vi "DCIMG to HDF5.vi"(4 "Time points":cluster{"Time Offset":i32, "Max length ":i32}={"Time Offset"=0, "Max length "=2147483647}, 5 "Chunk size":i32[](array[numeric])=[60, 256, 512], 6 "Frames per volume":i32=61, 7 "Channels":T1(array[cluster])=[{"X Offset"=0, "X Length"=512, "Y Offset"=0, "Y Length"=256, "Z Start"=0, "Z End"=60, "Z Stride"=1, "Name"="Far Red"}, {"X Offset"=512, "X Length"=512, "Y Offset"=0, "Y Length"=256, "Z Start"=0, "Z End"=60, "Z Stride"=1, "Name"="Red"}, {"X Offset"=1024, "X Length"=512, "Y Offset"=0, "Y Length"=256, "Z Start"=0, "Z End"=60, "Z Stride"=1, "Name"="Green"}], 8 "error in (no error)":errorcluster, 10 "Output path (*.h5)":path, 11 "Input path (*.dcimg)":path) -> (0 "error out":errorcluster)   [LabVIEW 2020]
uses:
  <vilib>/UPVI/lvhdf5/dataset.llb/LVH5D Operation.ctl
  <vilib>/Utility/miscctls.llb/LVRectTypeDef.ctl
  <vilib>/UPVI/lvhdf5/group.llb/H5G_obj_t.ctl
  <vilib>/Analysis/1siggen.llb/Ramp Pattern by Delta.vi
  <vilib>/UPVI/lvhdf5/utility.llb/Select HDF5 Dialog.vi
  <vilib>/UPVI/lvhdf5/utility.llb/Select HDF5 Dialog (Object Only).vi
  <vilib>/UPVI/lvhdf5/dataset.llb/Simple H5Dwrite (Variant).vi
  <vilib>/UPVI/lvhdf5/dataset.llb/Simple H5Dwrite.xnode
  <vilib>/UPVI/lvhdf5/library.llb/HDF5 Ref.ctl
  <vilib>/Analysis/NI_AALBase.lvlib
  <vilib>/UPVI/lvhdf5/identifier.llb/Not an HDF5 Refnum Constant.vi
  <vilib>/Utility/error.llb/Error Cluster From Error Code.vi
  <vilib>/UPVI/lvhdf5/dataset.llb/OpenCreateReplace Dataset by Element Type.vi
  <vilib>/UPVI/lvhdf5/dataspace.llb/H5Sselect_hyperslab.vi
  <vilib>/UPVI/lvhdf5/dataset.llb/H5Dwrite (Variant).vi
  <vilib>/UPVI/lvhdf5/dataset.llb/H5Dget_space.vi
  <vilib>/UPVI/lvhdf5/attribute.llb/private/LVH5AwriteWDTAttrs.vi
  <vilib>/UPVI/lvhdf5/dataspace.llb/H5Sclose.vi
  <vilib>/UPVI/lvhdf5/dataset.llb/H5Dclose.vi
  <vilib>/UPVI/lvhdf5/file.llb/OpenCreateReplace HDF5 File.vi
  <vilib>/UPVI/lvhdf5/file.llb/LVH5F Operation.ctl
  <vilib>/UPVI/lvhdf5/utility.llb/Select HDF5 Dialog (File and Object).vi
panel:
  out "total time (ms)":u32
  out "Progress":u8(slide) scale=0.0..100.0
  in  "Compression Level (0-disabled)":i32=1
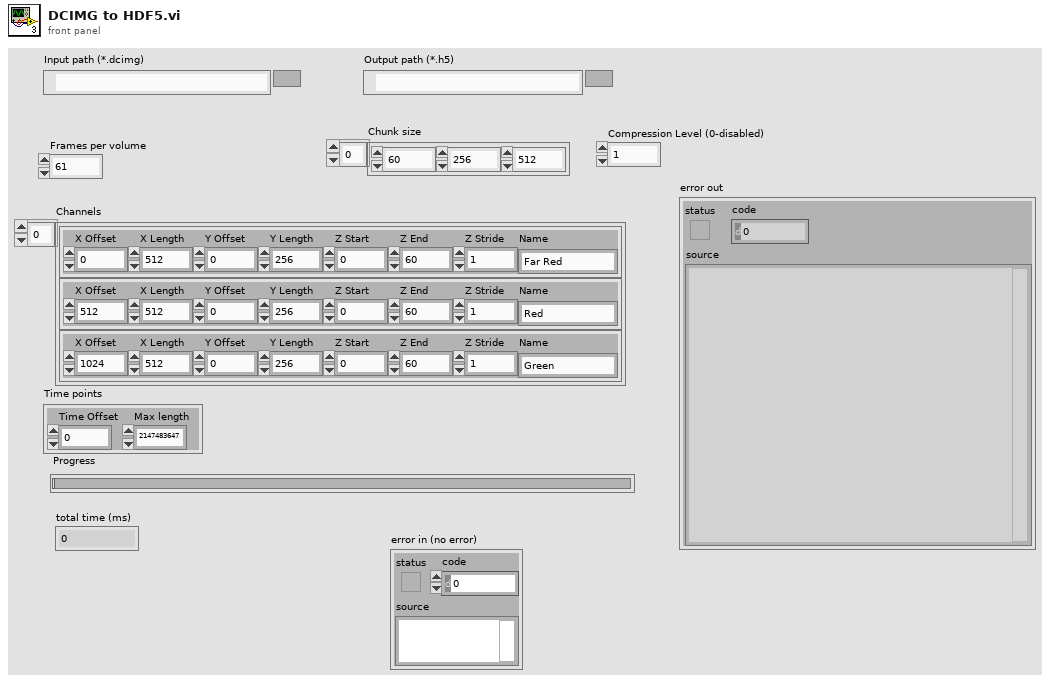
[diagram p1: front panel]
types:
  T1 = cluster{"X Offset":i32, "X Length":i32, "Y Offset":i32, "Y Length":i32, "Z Start":i32, "Z End":i32, "Z Stride":i32, "Name":string}[]
  T2 = typedef "HDF5 Ref.ctl" = refnum<k1>
  T3 = typedef "LVH5D Operation.ctl" = enum16{"open", "replace", "create", "open or create", "create or replace", "create or replace with confirmation"}
  T4 = typedef "LVRectTypeDef.ctl" = cluster{"Left":i16, "Top":i16, "Right":i16, "Bottom":i16}
  T5 = cluster{"Behavior":enum32{"Invalid", "Default", "Floating", "Floating/Auto-Hide", "Modal"}, "Position":T4, "Center":bool, "Title":string}
  T6 = typedef "LVH5F Operation.ctl" = enum16{"open", "open or create", "create or replace", "create or replace (with confirmation)", "create", "open (read only)"}
  T7 = typedef "H5G_obj_t.ctl" = i32
  T8 = cluster{"Object Types (any)":T7[], "Object Pattern":string}
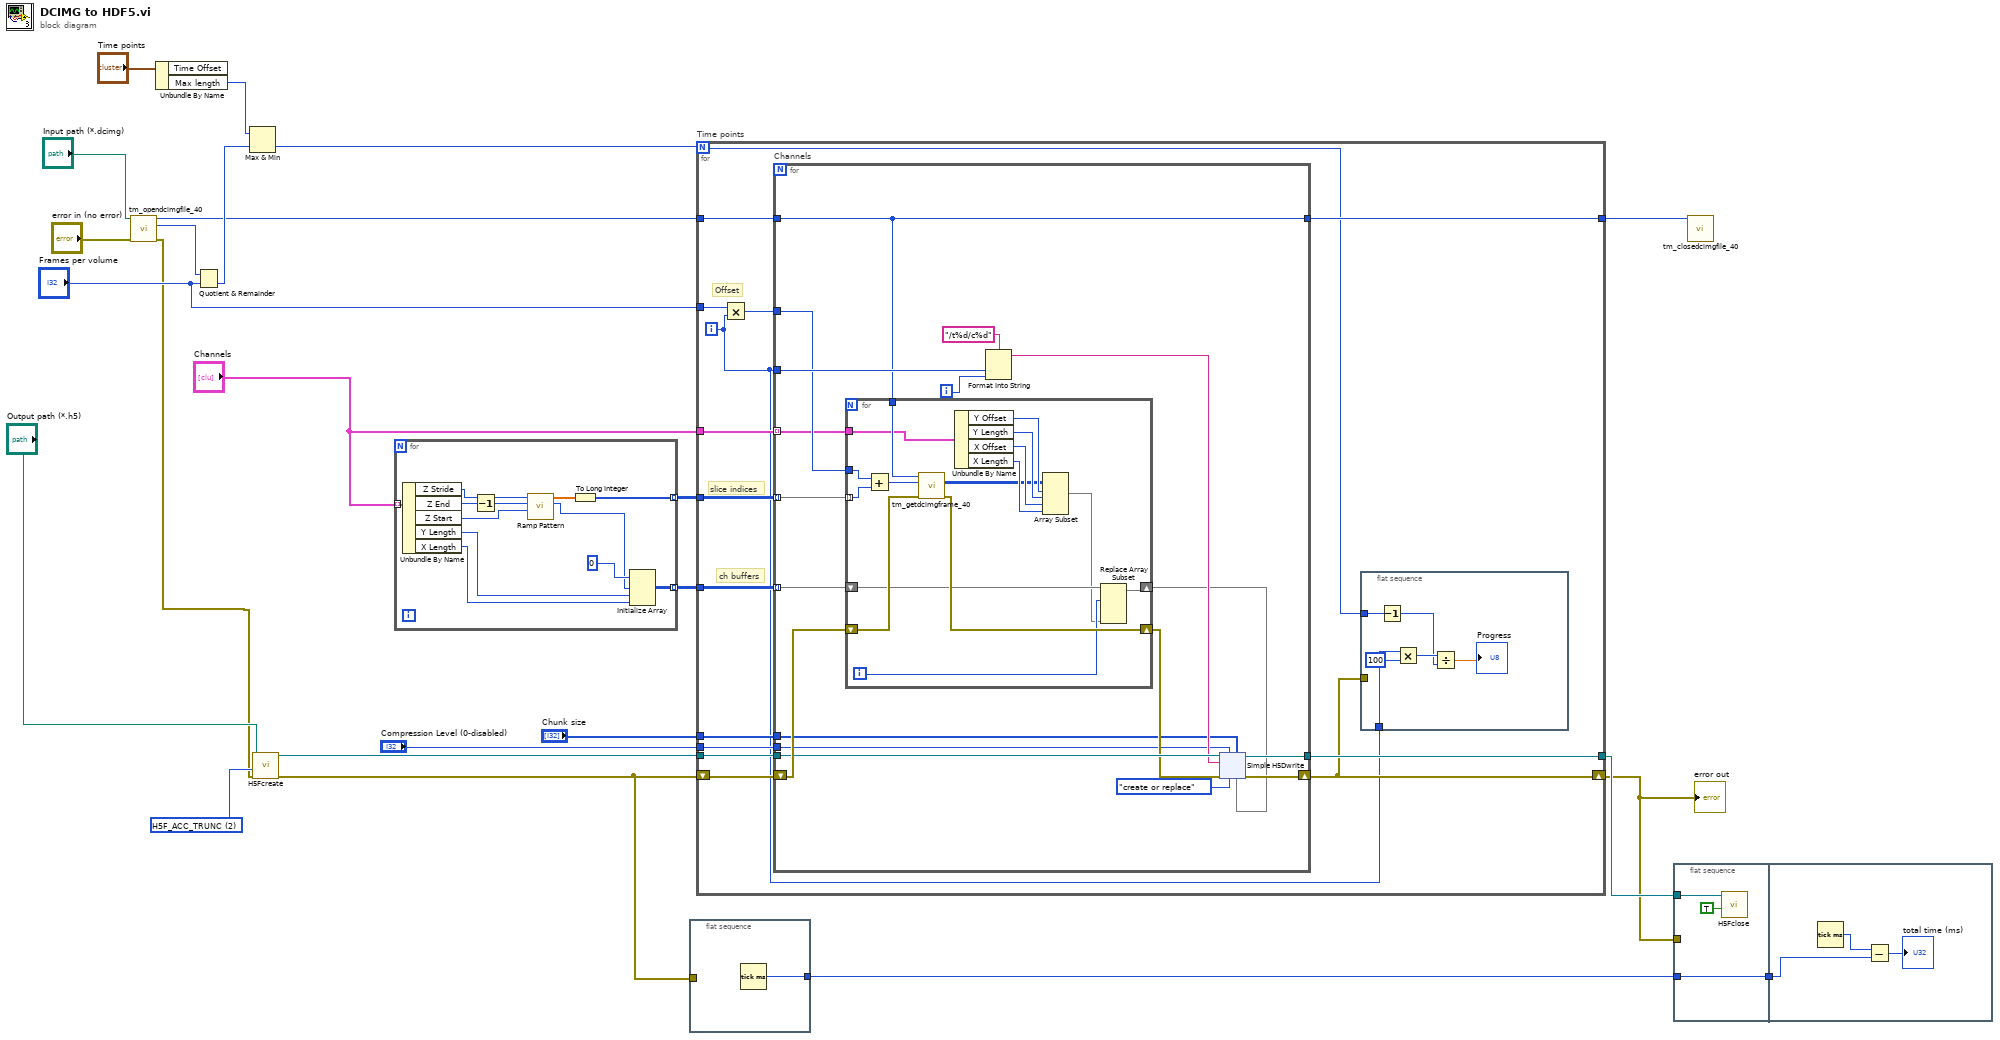
[diagram p0: block diagram]
diagram:
  w22 = u32 2 items=["H5F_ACC_TRUNC"=2, "H5F_ACC_EXCL"=4] ("flags")
  n1 = call <userlib>:"tm_opendcimgfile_40.vi"("error in (no error)"="error in (no error)", "Path"="Input path (*.dcimg)") -> ("error out"=w7:errorcluster, "Total Frames"=w21:i32, "File Handle"=w15:u32)  [unwired: 7 in]
  n2 = Unbundle By Name("Time points") -> ("Max length"=w17:i32)  [unwired: 1 out]
  n3 = Quotient & Remainder(x=w21, y="Frames per volume") -> (floor(x/y)=w19:i32)  [unwired: 1 out]
  n4 = Max & Min(x=w17, y=w19) -> (min(x,y)=w18:i32)  [unwired: 1 out]
  n5 = call <vilib>:"H5Fcreate.vi"("error in (no error)"=w7, "flags"=w22, "path"="Output path (*.h5)") -> ("error out"=w6:errorcluster, "HDF5 Ref"=w13:T2)  [unwired: 5 in]
  n6 = for {
    tunnel: "Channels" -> [w36] mode=indexing
    tunnel: [w33] -> w14 mode=indexing
    tunnel: [w31] -> w9 mode=indexing
    n7 = Unbundle By Name(w36) -> ("Z Stride"=w35:i32, "Z End"=w27:i32, "Z Start"=w25:i32, "Y Length"=w29:i32, "X Length"=w30:i32)
    n8 = Decrement(x=w27) -> (x-1=w26:i32)
    n9 = call-poly <vilib>:"Ramp Pattern.vi"("start"=w25, "end"=w26, "delta"=w35) -> ("samples"=w28:i32, "Ramp Pattern"=w34:dbl[])  [unwired: 6 in, 1 out]
    n10 = To Long Integer(number=w34) -> (32bit integer=w33:i32[])
    n11 = Initialize Array(u16 0 ("element"), w28, w29, w30) -> (w31:u16[][][])
  }
  n12 = flat-sequence {
    tunnel: w6 -> [_]
    tunnel: [w37] -> w5
    frame #0 {
      n13 = Tick Count (ms)() -> (millisecond timer value=w37:u32)
    }
  }
  n14 = for "Time points" {
    N: w18 -> [w39]
    tunnel: "Channels" -> [w52]
    tunnel: "Frames per volume" -> [w51]
    tunnel: w15 -> [w50]
    tunnel: w14 -> [w48]
    tunnel: w13 -> [w47]
    tunnel: "Chunk size" -> [w45]
    tunnel: "Compression Level (0-disabled)" -> [w44]
    tunnel: w9 -> [w43]
    shift-right: [w40] -> w2
    shift-left: w6 -> [w46]
    tunnel: [w42] -> w8
    tunnel: [w41] -> w3
    i -> [w38]
    # "slice indices"
    # "ch buffers"
    # "Offset"
    n15 = Multiply(x=w51, y=w38) -> (x*y=w49:i32)
    n16 = for "Channels" {
      tunnel: w52 -> [w68] mode=indexing
      tunnel: w50 -> [w69]
      tunnel: w49 -> [w72]
      tunnel: w48 -> [w73] mode=indexing
      tunnel: w38 -> [w74]
      tunnel: w47 -> [w67]
      tunnel: w45 -> [w59]
      tunnel: w44 -> [w63]
      tunnel: w43 -> [w71] mode=indexing
      shift-right: [w62] -> w40
      shift-left: w46 -> [w70]
      tunnel: [w69] -> w42
      tunnel: [w61] -> w41
      i -> [w75]
      n17 = for {
        tunnel: w73 -> [w293] mode=indexing
        tunnel: w72 -> [w294]
        shift-right: [w289] -> w65
        shift-left: w70 -> [w292]
        tunnel: w69 -> [w290]
        tunnel: w68 -> [w288]
        shift-right: [w282] -> w60
        shift-left: w71 -> [w283]
        i -> [w281]
        n18 = Add(x=w294, y=w293) -> (x+y=w291:i32)
        n19 = call <userlib>:"tm_getdcimgframe_40.vi"("error in (no error)"=w292, "Frame Index"=w291, "File Handle in"=w290) -> ("error out"=w289:errorcluster, "Data"=w280:u16[][])  [unwired: 5 in, 2 out]
        n20 = Unbundle By Name(w288) -> ("Y Offset"=w284:i32, "Y Length"=w285:i32, "X Offset"=w286:i32, "X Length"=w287:i32)
        n21 = Array Subset(array=w280, index (row)=w284, length (row)=w285, index (col)=w286, length (col)=w287) -> (w279:u16[][])
        n22 = Replace Array Subset(array=w283, new element=w279, index (dim 0)=w281) -> (w282:u16[][][])  [unwired: 2 in]
      }
      n23 = Format Into String(format string="/t%d/c%d", w74, w75) -> (resulting string=w66:string)  [unwired: 2 in, 1 out]
      n24 = xnode "Simple H5Dwrite"("Chunk size"=w59, "Compression Level (0-disabled)"=w63, "Dataset Path"=w66, "error in (no error)"=w65, "operation (open or create)"=LVH5D_Operation."create or replace", "HDF5 Path or Ref"=w67, "Data"=w60) -> ("HDF5 Ref out"=w61:T2, "error out"=w62:errorcluster)  [unwired: 1 in, 1 out]
    }
    n25 = flat-sequence {
      tunnel: w40 -> [_]
      tunnel: w39 -> [w54]
      tunnel: w38 -> [w58]
      frame #0 {
        n26 = Decrement(x=w54) -> (x-1=w53:i32)
        n27 = Multiply(x=w58, y=100) -> (x*y=w56:i32)
        n28 = Divide(x=w56, y=w53) -> (x/y=→"Progress":dbl)
      }
    }
  }
  "error out" <- w2
  n29 = flat-sequence {
    tunnel: w5 -> [w297]
    tunnel: [w297] -> w4
    tunnel: w3 -> [w295]
    tunnel: w2 -> [_]
    tunnel: w4 -> [w299]
    frame #0 {
      n30 = call <vilib>:"H5Fclose.vi"("Force Close (F)"=TRUE, "HDF5 Ref"=w295) -> ()  [unwired: 7 in, 1 out]
    }
    frame #1 {
      n31 = Tick Count (ms)() -> (millisecond timer value=w300:u32)
      n32 = Subtract(x=w300, y=w299) -> (x-y=→"total time (ms)":u32)
    }
  }
  n33 = call <userlib>:"tm_closedcimgfile_40.vi"("File Handle"=w8) -> ()  [unwired: 10 in, 1 out]
